vi "Synth_Step_Size.vi"(11 "Step Size":string) -> ()   [LabVIEW 2024]
uses:
  Serial Port.vi
  <vilib>/Instr/_visa.llb/VISA Configure Serial Port (Instr).vi
panel:
  out "Combo Box":string(combo)
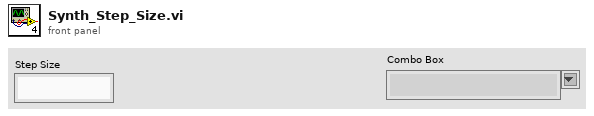
[diagram p1: front panel]
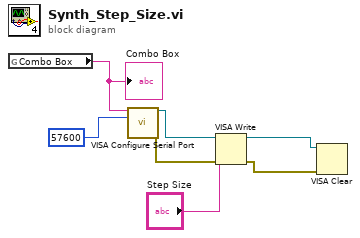
[diagram p0: block diagram]
diagram:
  n1 = global read "Serial Port.vi" "Combo Box"() -> (w1:string)
  "Combo Box" <- w1
  n2 = call-poly "VISA Configure Serial Port"("VISA resource name"=w1, "baud rate (9600)"=u32 57600) -> ("VISA resource name out"=w6:refnum<visa-resource-name>, "error out"=w3:errorcluster)  [unwired: 12 in]
  n3 = VISA Write(VISA resource name=w6, write buffer="Step Size", error in (no error)=w3) -> (VISA resource name out=w4:refnum<visa-resource-name>, error out=w2:errorcluster)  [unwired: 1 out]
  n4 = VISA Clear(VISA resource name=w4, error in (no error)=w2) -> ()  [unwired: 2 out]
